vi "Open Handle.vi"(6 "verify server(true)":bool=TRUE, 7 "cookie file":path, 8 "error in (no error)":errorcluster, 9 "password":string, 10 "username":string, 11 "HTTP Client Abstract in":refnum<class "Abstract HTTP Client.lvclass">) -> (0 "error out":errorcluster, 3 "HTTP Client Abstract out":refnum<class "Abstract HTTP Client.lvclass">)   [LabVIEW 2020, in "HTTP Client Abstract.lvlib" / "Abstract HTTP Client.lvclass"]
uses:
  Abstract HTTP Client.lvclass
  LabVIEW HTTP Client/LabVIEW HTTP Client.lvclass
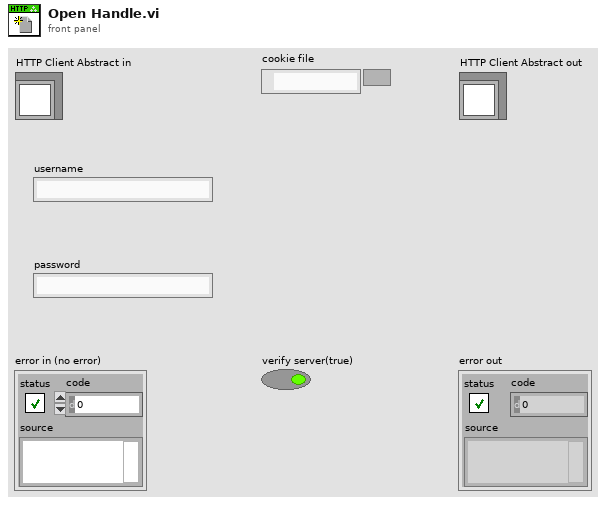
[diagram p1: front panel]
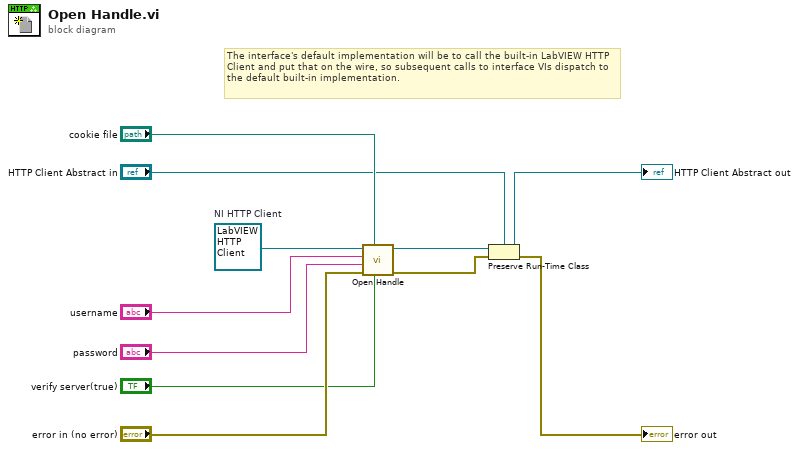
[diagram p0: block diagram]
diagram:
  w11 = refnum<class "LabVIEW HTTP Client.lvclass"> refnum  # NI HTTP Client
  # "The interface's default implementation will be to call the built-in LabVIEW HTTP Client and put that on the wire, so subsequent calls to interface VIs dispatch to the default built-in implementation."
  n1 = call-dynamic "Open Handle.vi"("verify server(true)"="verify server(true)", "cookie file"="cookie file", "error in (no error)"="error in (no error)", "password"="password", "username"="username", "HTTP Client Base in"=w11) -> ("error out"=w3:errorcluster, "HTTP Client Base out"=w6:refnum<class "LabVIEW HTTP Client.lvclass">)  [unwired: 4 in]
  n2 = Preserve Run-Time Class(object in=w6, error in=w3, 2:"HTTP Client Abstract in") -> (object out=→"HTTP Client Abstract out":refnum<class "Abstract HTTP Client.lvclass">, error out=→"error out":errorcluster)
